vi "TxRollback_Core.vi"(8 "error in (no error)":errorcluster, 11 "DBC in":refnum<class "DBC.lvclass">) -> (0 "error out":errorcluster, 3 "DBC out":refnum<class "DBC.lvclass">)   [LabVIEW 2020, in "ORM_pgsql_jdp.lvlib" / "DBC.lvclass"]
uses:
  DBC.lvclass
  DBC.lvclass/DBC.ctl
  <vilib>/JDP Science/PostgreSQL Library/Connection/Execute (no results).vi
  <vilib>/JDP Science/PostgreSQL Library/Connection/Execute (Return first result with rows).vi
  <vilib>/JDP Science/PostgreSQL Library/Connection/Execute Single Statement (String Parameters).vi
  <vilib>/JDP Science/PostgreSQL Library/Result/Clear.vi
  <vilib>/JDP Science/PostgreSQL Library/Connection/PQ Connection.lvclass
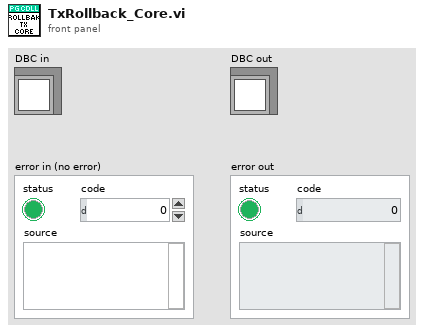
[diagram p1: front panel]
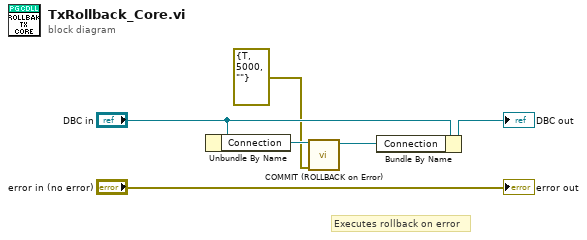
[diagram p0: block diagram]
diagram:
  # "Executes rollback on error"
  n1 = Unbundle By Name("DBC in") -> ("Connection"=w4:refnum<class "PQ Connection.lvclass">)
  n2 = call <vilib>:"COMMIT (ROLLBACK on Error).vi"("error in (no error)"=errorcluster {"status"=TRUE, "code"=5000, "source"=""}, "PQ Connection in"=w4) -> ("PQ Connection out"=w1:refnum<class "PQ Connection.lvclass">)  [unwired: 8 in, 1 out]
  n3 = Bundle By Name(cluster="DBC in", "Connection"=w1) -> (→"DBC out":refnum<class "DBC.lvclass">)
  "error out" <- "error in (no error)"
